vi "Open Modbus.vi"(8 "error in (no error)":errorcluster, 11 "Modbus_TCP in":refnum<class "Modbus_TCP.lvclass">) -> (0 "error out":errorcluster, 3 "Modbus_TCP out":refnum<class "Modbus_TCP.lvclass">)   [LabVIEW 2021, in "Modbus_TCP.lvclass"]
uses:
  Modbus_TCP.lvclass
  C:/Users/lincoln.lucio/Documents/Lincoln/Documentos Pessoais/meus docs/Projetos pessoais/Projeto Sciranda/projeto_versioned/sciranda/Modbus_Master/Modbus_Master.lvclass
  Modbus_Master/Modbus_Master.lvclass/Modbus_Master.ctl
  Modbus_TCP.lvclass/Modbus_TCP.ctl
  <vilib>/NI/Modbus Library/API/Modbus API.lvclass/Modbus API.ctl
  <vilib>/NI/Modbus Library/Transmission Data Unit/Transmission Data Unit.lvclass/Transmission Data Unit.ctl
  Modbus_Master/Accessor VIs/Read Timeout(ms).vi
  Modbus_Master/Accessor VIs/Read unit ID.vi
  Modbus_Master/Accessor VIs/Write master instance.vi
  <vilib>/NI/Modbus Library/Transmission Data Unit/Write Unit ID.vi
  <vilib>/NI/Modbus Library/API/Read Transmission Data Unit.vi
  <vilib>/NI/Modbus Library/API/Write Transmission Data Unit.vi
  <vilib>/NI/Modbus Library/API/Master/Modbus Master.lvclass
  C:/Program Files/National Instruments/LabVIEW 2021/vi.lib/NI/Modbus Library/API/Modbus API.lvclass
  <vilib>/NI/Modbus Library/API/Wrapper/Create TCP Master.vi
  <vilib>/NI/Modbus Library/API/Wrapper/API Main.lvlib
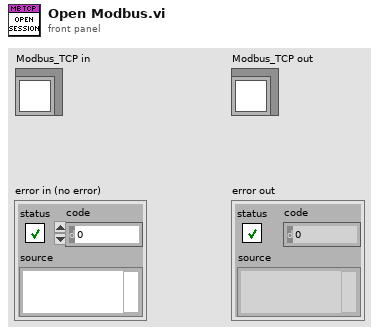
[diagram p1: front panel]
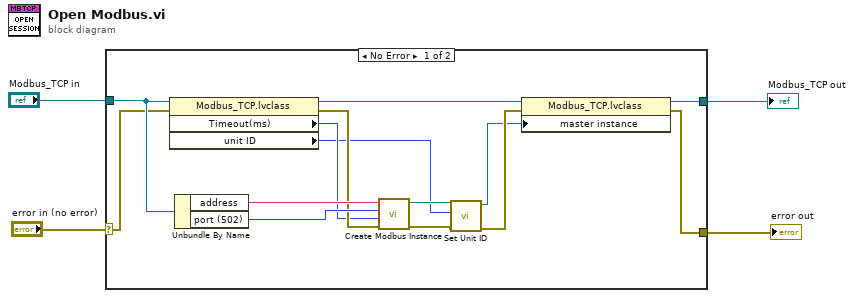
[diagram p0: block diagram]
diagram:
  n1 = case shown="No Error" "error in (no error)" {
    selector: "error in (no error)" -> [w11 w20]
    tunnel: [w16 w19] -> w4
    tunnel: "Modbus_TCP in" -> [w15 w19]
    tunnel: [w12 w20] -> w2
    frame No Error {
      n2 = property class="Modbus_TCP.lvclass"(reference=w15, error in=w11) -> (reference out=w14:refnum<class "Modbus_TCP.lvclass">, error out=w13:errorcluster, "Timeout(ms)"=w10:i32, "unit ID"=w5:u8)
      n3 = Unbundle By Name(w15) -> ("address"=w18:string, "port (502)"=w17:u16)
      n4 = call-poly <vilib>:"Create Modbus Instance.vi"("error in"=w13, "connect timeout ms"=w10, "port (502)"=w17, "address"=w18) -> ("error out"=w8:errorcluster, "TCP master instance"=w9:refnum<class "Modbus Master.lvclass">)  [unwired: 6 in]
      n5 = call <vilib>:"Set Unit ID.vi"("error in"=w8, "unit ID"=w5, "Modbus master in"=w9) -> ("error out"=w7:errorcluster, "Modbus master out"=w6:refnum<class "Modbus Master.lvclass">)  [unwired: 7 in]
      n6 = property class="Modbus_TCP.lvclass"(reference=w14, error in=w7, "master instance"=w6) -> (reference out=w16:refnum<class "Modbus_TCP.lvclass">, error out=w12:errorcluster)
    }
    frame Error {
    }
  }
  "error out" <- w2
  "Modbus_TCP out" <- w4
